vi "Write IFD.vi"(0 "Byte Stream File in":refnum<file>, 1 "Additional Named Tags":cluster{"name":string, "Variant":variant}[](array[cluster]), 2 "Additional Tags":T4(array[cluster]), 3 "byte order (0:big-endian, network order)":T9(ring), 5 "IFD Offset Position":i64 format="%x", 9 "Offset":i64, 11 "error in":errorcluster, 12 "IFD Baseline":T8 {"SampleFormat" items=["UINT"=1, "INT"=2, "FP"=3, "VOID"=4, "COMPLEXINT"=5, "COMPLEXFP"=6]; "NewSubFileType" items=["FILETYPE_REDUCEDIMAGE"=1, "FILETYPE_PAGE"=2, "FILETYPE_MASK"=4]; "Compression" items=["COMPRESSION_NONE"=1, "COMPRESSION_CCITTRLE"=2, "COMPRESSION_CCITTFAX3"=3, "COMPRESSION_CCITTFAX4"=4, "COMPRESSION_LZW"=5, "COMPRESSION_OJPEG"=6, "COMPRESSION_JPEG"=7, "COMPRESSION_NEXT"=32766, "COMPRESSION_CCITTRLEW"=32771, "COMPRESSION_PACKBITS"=32773, "COMPRESSION_THUNDERSCAN"=32809, "COMPRESSION_IT8CTPAD"=32895, "COMPRESSION_IT8LW"=32896, "COMPRESSION_IT8MP"=32897, "COMPRESSION_IT8BL"=32898, "COMPRESSION_PIXARFILM"=32908, "COMPRESSION_PIXARLOG"=32909, "COMPRESSION_DEFLATE"=32946, "COMPRESSION_ADOBE_DEFLATE"=8, "COMPRESSION_DSC"=32947, "COMPRESSION_JBIG"=34661, "COMPRESSION_SGILOG"=34676, "COMPRESSION_SGILOG24"=34677, "COMPRESSION_JP2000"=34712]; "PhotometricInterpretation" items=["PHOTOMETRIC_MINISWHITE"=0, "PHOTOMETRIC_MINISBLACK"=1, "PHOTOMETRIC_RGB"=2, "PHOTOMETRIC_PALETTE"=3, "PHOTOMETRIC_MASK"=4, "PHOTOMETRIC_SEPARATED"=5, "PHOTOMETRIC_YCBCR"=6, "PHOTOMETRIC_CIELAB"=8, "PHOTOMETRIC_ICCLAB"=9, "PHOTOMETRIC_ITULAB"=10, "PHOTOMETRIC_LOGL"=32844, "PHOTOMETRIC_LOGLUV"=32845, "CFA"=32803, "LinearRaw"=34892, "DEPTH"=51177]; "ResolutionUnit" items=["RESUNIT_NONE"=1, "RESUNIT_INCH"=2, "RESUNIT_CENTIMETER"=3]}, 14 "Details":T5={"ImageDescription"="", "XResolution"=0.0, "YResolution"=0.0, "ResolutionUnit"=enum."Inch", "PhotometricInterpretation"=0, "Compression"=enum."None", "PageName"="", "DocumentName"=""} {"PhotometricInterpretation" items=["PHOTOMETRIC_MINISWHITE"=0, "PHOTOMETRIC_MINISBLACK"=1, "PHOTOMETRIC_RGB"=2, "PHOTOMETRIC_PALETTE"=3, "PHOTOMETRIC_MASK"=4, "PHOTOMETRIC_SEPARATED"=5, "PHOTOMETRIC_YCBCR"=6, "PHOTOMETRIC_CIELAB"=8, "PHOTOMETRIC_ICCLAB"=9, "PHOTOMETRIC_ITULAB"=10, "PHOTOMETRIC_LOGL"=32844, "PHOTOMETRIC_LOGLUV"=32845, "CFA"=32803, "LinearRaw"=34892, "DEPTH"=51177]}) -> (4 "refnum out":refnum<file>, 6 "Next IFD Offset Position":i64 format="%x", 10 "Next Offset":i64, 15 "error out":errorcluster)   [LabVIEW 2020, in "LV Tiff.lvlib"]
uses:
  LV Tiff.lvlib
  Baseline Tags 1.ctl
  Tiff Tag.ctl
  Tiff Tags.ctl
  Tiff Data Type.ctl
  Tiff Page Details.ctl
  <vilib>/Utility/Data Type/Type Definitions/Data Type.ctl
  13cce788-e93b-439c-a4f4-f02fbe767664.vi
  de296096-4773-46d0-ada0-82523eb18cea.vi
  <vilib>/Comparison/Less/Less Functor/Less Functor.lvclass
  <vilib>/Utility/Data Type/NI_Data Type.lvlib
panel:
  out "sorted array":T3(array[cluster])
  out "Written Tags":T6[](array[typedef]) {"TagID" items=["NewSubfileType"=254, "ImageWidth"=256, "ImageLength"=257, "BitsPerSample"=258, "Compression"=259, "PhotometricInterpretation"=262, "StripOffsets"=273, "SamplesPerPixel"=277, "RowsPerStrip"=278, "StripByteCounts"=279, "XResolution"=282, "YResolution"=283, "ResolutionUnit"=296, "ColorMap"=320, "PlanarConfiguration"=284, "YCbCrCoefficients"=529, "YCbCrSubSampling"=530, "YCbCrPositioning"=531, "ReferenceBlackWhite"=532, "BadFaxLines"=326, "CleanFaxData"=327, "ConsecutiveBadFaxLines"=328, "SampleFormat"=339]}
  out "This IFD Position":u32
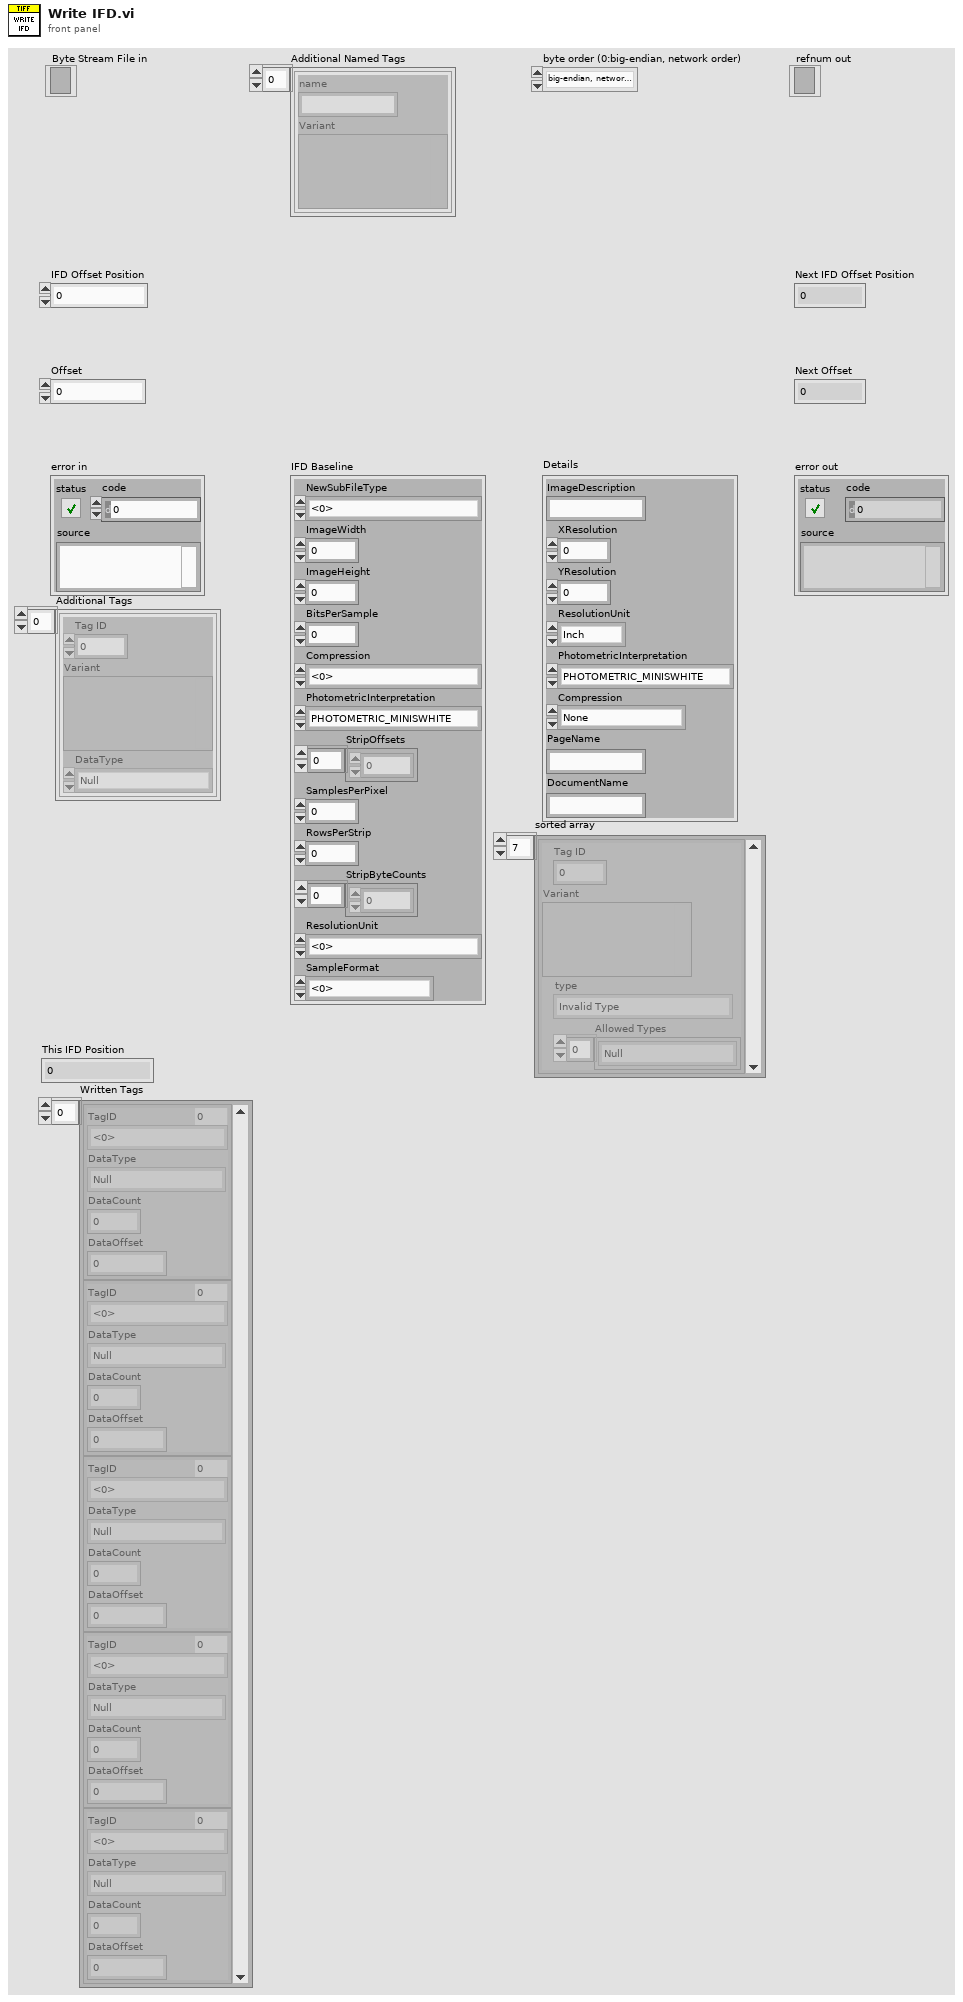
[diagram p1: front panel]
types:
  T1 = typedef "NI_Data Type.lvlib/Data Type.ctl" = enum8{"Invalid Type", "Void", "I8", "I16", "I32", "I64", "U8", "U16", "U32", "U64", "Single Float", "Double Float", "Extended Float", "Single Complex", "Double Complex", "Extended Complex", "Enum U8", "Enum U16", "Enum U32", "Enum U64", "Single Float With Unit", "Double Float With Unit", "Extended Float With Unit", "Single Complex with Unit", "Double Complex with Unit", "Extended Complex with Unit", "Boolean", "String", "Path", "Picture", "Tag", "Array", "Cluster", "Variant", "LV Variant", "Waveform", "Timestamp", "Digital Waveform", "Digital Data", "ExpressData", "Refnum", "External Data", "VI", "Poly VI", "LabVIEW Class Instance", "Fixed Point", "Set Collection", "Map Collection"}
  T2 = typedef "LV Tiff.lvlib/Tiff Data Type.ctl" = enum16{"Null", "BYTE", "ASCII", "SHORT", "LONG", "RATIONAL", "SBYTE", "UNDEFINE", "SSHORT", "SLONG", "SRATIONAL", "FLOAT", "DOUBLE"}
  T3 = cluster{"Tag ID":u32, "Variant":variant, "type":T1, "Allowed Types":T2[]}[]
  T4 = cluster{"Tag ID":u32, "Variant":variant, "DataType":T2}[]
  T5 = typedef "LV Tiff.lvlib/Tiff Page Details.ctl" = cluster{"ImageDescription":string, "XResolution":dbl, "YResolution":dbl, "ResolutionUnit":enum16{"None", "Inch", "Centimeter"}, "PhotometricInterpretation":u16, "Compression":enum16{"None", "Deflate", "JPEG"}, "PageName":string, "DocumentName":string}
  T6 = typedef "LV Tiff.lvlib/Tiff Tag.ctl" = cluster{"TagID":T7, "DataType":T2, "DataCount":u32, "DataOffset":u32}
  T7 = typedef "LV Tiff.lvlib/Tiff Tags.ctl" = u16
  T8 = typedef "LV Tiff.lvlib/Baseline Tags 1.ctl" = cluster{"NewSubFileType":u32, "ImageWidth":u32, "ImageHeight":u32, "BitsPerSample":u16, "Compression":u16, "PhotometricInterpretation":u16, "StripOffsets":u32[], "SamplesPerPixel":u16, "RowsPerStrip":u32, "StripByteCounts":u32[], "ResolutionUnit":u16, "SampleFormat":u16}
  T9 = enum16{"big-endian, network order", "native, host order", "little-endian"}
  T10 = map{string, cluster{"Tag ID":u32, "Allowed Types":T2[]}}
  T11 = cluster{"Tag ID":u32, "Variant":variant, "type":T1, T2[]}
  T12 = cluster{"name":string, "Variant":variant, "type":T1}
  T13 = cluster{"name":string, "Variant":variant, "type":T1}[]
  T14 = cluster{"Tag ID":u32, "Variant":variant, "type":T1, "Allowed Types":T2[]}
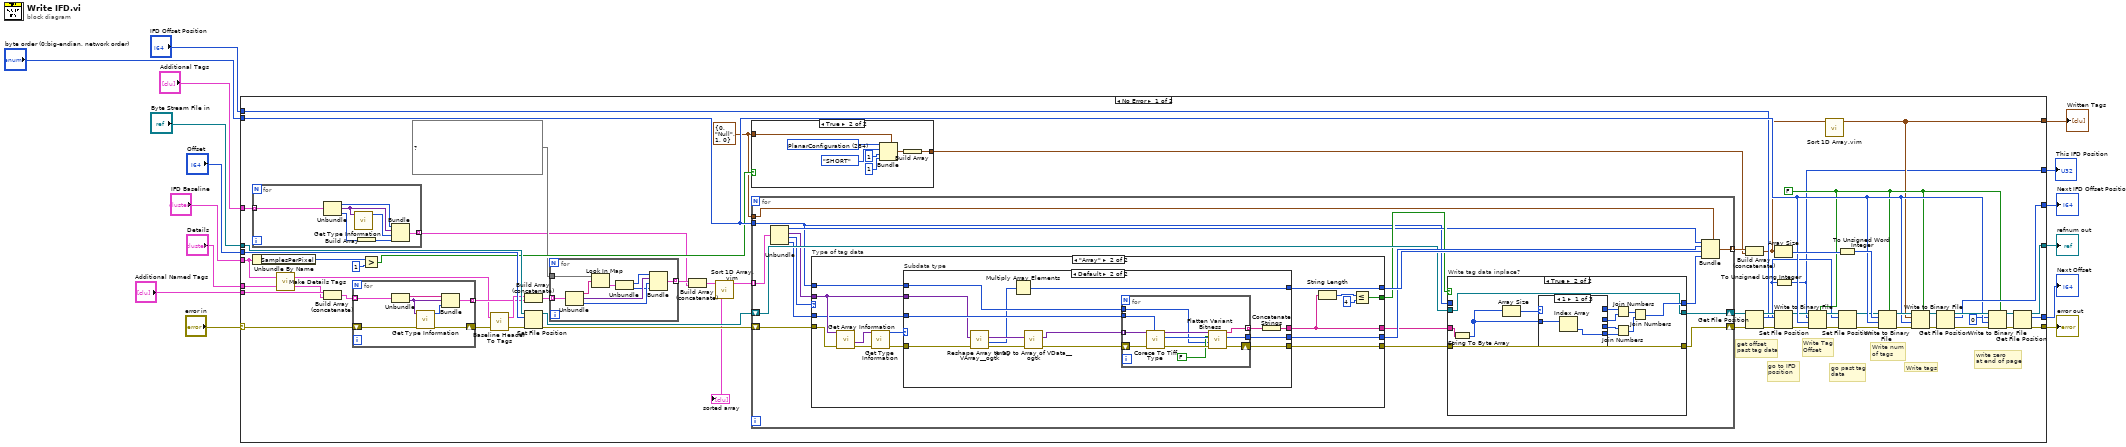
[diagram p0: block diagram]
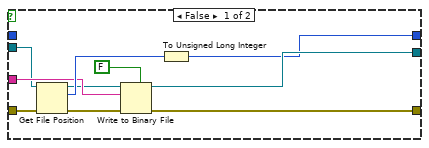
[diagram p3: hidden frame]
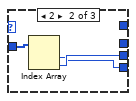
[diagram p4: hidden frame]
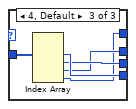
[diagram p5: hidden frame]
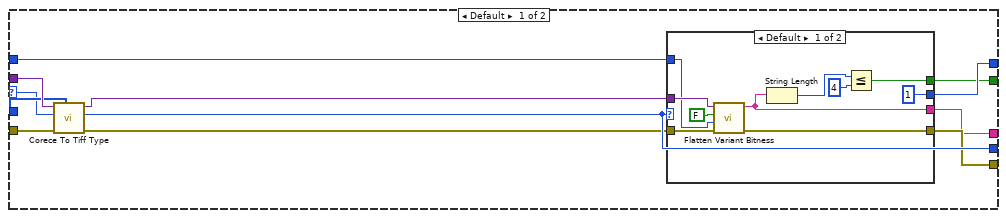
[diagram p6: hidden frame]
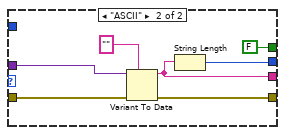
[diagram p7: hidden frame]
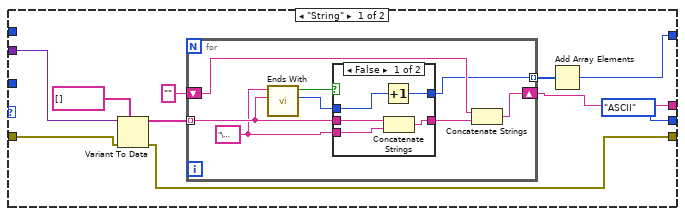
[diagram p8: hidden frame]
diagram:
  n1 = case shown="No Error" "error in" {
    selector: "error in" -> [w38 w250]
    tunnel: "Offset" -> [w75 _]
    tunnel: "Byte Stream File in" -> [w73 w249]
    tunnel: "IFD Baseline" -> [w27 _]
    tunnel: [w63 _] -> w12
    tunnel: [w59 w250] -> w10
    tunnel: [w57 w249] -> w9
    tunnel: [w56 _] -> w8
    tunnel: "byte order (0:big-endian, network order)" -> [w52 _]
    tunnel: "IFD Offset Position" -> [w47 _]
    tunnel: "Additional Named Tags" -> [w40 _]
    tunnel: "Details" -> [w28 _]
    tunnel: "Additional Tags" -> [w22 _]
    tunnel: [w17 _] -> w2
    tunnel: [w16 _] -> w1
    frame No Error {
      w51 = FALSE ("prepend array or string size? (T)")
      w30 = T6 {"TagID"=0, "DataType"=enum."Null", "DataCount"=1, "DataOffset"=0}
      # "write zero\nat end of page"
      # "Write tags"
      # "Write num\nof tags"
      # "go past tag\ndata"
      # "Write Tag\nOffset"
      # "go to IFD position"
      # "get offset\npast tag data"
      n2 = for {
        tunnel: w22 -> [w82] mode=indexing
        tunnel: [w78] -> w21 mode=indexing
        n3 = Unbundle(w82) -> ("Tag ID"=w81:u32, "Variant"=w80:variant, "DataType"=w77:T2)
        n4 = call <vilib>:"Get Type Information.vi"("variant"=w80) -> ("type"=w79:T1)  [unwired: 6 in, 4 out]
        n5 = Build Array(w77) -> (w76:T2[])
        n6 = Bundle("Tag ID"=w81, "Variant"=w80, "type"=w79, w76) -> (w78:T11)  [unwired: 1 in]
      }
      n7 = Unbundle By Name(w27) -> ("SamplesPerPixel"=w33:u16)
      n8 = call "Make Details Tags.vi"("Details"=w28, "IFD Baseline"=w27) -> ("Tags"=w35:cluster{"name":string, "Variant":variant}[], "Modified IFD Baseline"=w26:T8)
      n9 = Build Array (concatenate)(w40, w35) -> (w36:cluster{"name":string, "Variant":variant}[])
      n10 = for {
        tunnel: w36 -> [w105] mode=indexing
        tunnel: [w101] -> w39 mode=indexing
        shift-right: [w99] -> w37
        shift-left: w38 -> [w100]
        n11 = Unbundle(w105) -> ("name"=w104:string, "Variant"=w103:variant)
        n12 = call <vilib>:"Get Type Information.vi"("error in (no error)"=w100, "variant"=w103) -> ("error out"=w99:errorcluster, "type"=w102:T1)  [unwired: 5 in, 3 out]
        n13 = Bundle("name"=w104, "Variant"=w103, "type"=w102) -> (w101:T12)  [unwired: 1 in]
      }
      n14 = Greater?(x=w33, y=u16 1) -> (0:w32:bool)
      n15 = call "Baseline Header To Tags.vi"("error in"=w37, "IFD Baseline"=w26) -> ("error out"=w42:errorcluster, "Tags"=w41:T13)
      n16 = Build Array (concatenate)(w41, w39) -> (w24:T13)
      n17 = Set File Position(offset (in bytes) (0)=w75, refnum=w73, error in=w42) -> (refnum out=w74:refnum<file>, error out=w61:errorcluster)  [unwired: 1 in]
      n18 = for {
        tunnel: T10 {"Artist"={"Tag ID"=315, "Allowed Types"=[enum."ASCII"]}, "BadFaxLines"={"Tag ID"=326, "Allowed Types"=[enum."SHORT", enum."LONG"]}, "BitsPerSample"={"Tag ID"=258, "Allowed Types"=[enum."SHORT"]}, "BlackIsZero"={"Tag ID"=1, "Allowed Types"=[]}, "CCITT 1D"={"Tag ID"=2, "Allowed Types"=[]}, "CCITT Group 3"={"Tag ID"=3, "Allowed Types"=[]}, "CCITT Group 4"={"Tag ID"=4, "Allowed Types"=[]}, "CIELab"={"Tag ID"=8, "Allowed Types"=[]}, "CMYK"={"Tag ID"=5, "Allowed Types"=[]}, "CellLength"={"Tag ID"=265, "Allowed Types"=[enum."SHORT"]}, "CellWidth"={"Tag ID"=264, "Allowed Types"=[enum."SHORT"]}, "CleanFaxData"={"Tag ID"=327, "Allowed Types"=[enum."SHORT"]}, "ColorMap"={"Tag ID"=320, "Allowed Types"=[enum."SHORT"]}, "ColorResponseCurve"={"Tag ID"=301, "Allowed Types"=[enum."SHORT"]}, "ColorResponseUnit"={"Tag ID"=300, "Allowed Types"=[enum."SHORT"]}, "Compression"={"Tag ID"=259, "Allowed Types"=[enum."SHORT"]}, "ConsecutiveBadFaxLines"={"Tag ID"=328, "Allowed Types"=[enum."LONG", enum."SHORT"]}, "Copyright"={"Tag ID"=33432, "Allowed Types"=[enum."ASCII"]}, "DateTime"={"Tag ID"=306, "Allowed Types"=[enum."ASCII"]}, "DocumentName"={"Tag ID"=269, "Allowed Types"=[enum."ASCII"]}, "DotRange"={"Tag ID"=336, "Allowed Types"=[enum."BYTE", enum."SHORT"]}, "ExtraSamples"={"Tag ID"=338, "Allowed Types"=[enum."BYTE"]}, "FillOrder"={"Tag ID"=266, "Allowed Types"=[enum."SHORT"]}, "FreeByteCounts"={"Tag ID"=289, "Allowed Types"=[enum."LONG"]}, "FreeOffsets"={"Tag ID"=288, "Allowed Types"=[enum."LONG"]}, "GrayResponseCurve"={"Tag ID"=291, "Allowed Types"=[enum."SHORT"]}, "GrayResponseUnit"={"Tag ID"=290, "Allowed Types"=[enum."SHORT"]}, "HalftoneHints"={"Tag ID"=321, "Allowed Types"=[enum."SHORT"]}, "HostComputer"={"Tag ID"=316, "Allowed Types"=[enum."ASCII"]}, "ImageDescription"={"Tag ID"=270, "Allowed Types"=[enum."ASCII"]}, "ImageHeight"={"Tag ID"=257, "Allowed Types"=[enum."SHORT", enum."LONG"]}, "ImageWidth"={"Tag ID"=256, "Allowed Types"=[enum."SHORT", enum."LONG"]}, "InkNames"={"Tag ID"=333, "Allowed Types"=[enum."ASCII"]}, "InkSet"={"Tag ID"=332, "Allowed Types"=[enum."SHORT"]}, "JPEG"={"Tag ID"=6, "Allowed Types"=[]}, "JPEGACTTables"={"Tag ID"=521, "Allowed Types"=[enum."LONG"]}, "JPEGDCTTables"={"Tag ID"=520, "Allowed Types"=[enum."LONG"]}, "JPEGInterchangeFormat"={"Tag ID"=513, "Allowed Types"=[enum."LONG"]}, "JPEGInterchangeFormatLength"={"Tag ID"=514, "Allowed Types"=[enum."LONG"]}, "JPEGLosslessPredictors"={"Tag ID"=517, "Allowed Types"=[enum."SHORT"]}, "JPEGPointTransforms"={"Tag ID"=518, "Allowed Types"=[enum."SHORT"]}, "JPEGProc"={"Tag ID"=512, "Allowed Types"=[enum."SHORT"]}, "JPEGQTables"={"Tag ID"=519, "Allowed Types"=[enum."LONG"]}, "JPEGRestartInterval"={"Tag ID"=515, "Allowed Types"=[enum."SHORT"]}, "LZW"={"Tag ID"=5, "Allowed Types"=[]}, "Make"={"Tag ID"=271, "Allowed Types"=[enum."ASCII"]}, "MaxSampleValue"={"Tag ID"=281, "Allowed Types"=[enum."SHORT"]}, "MinSampleValue"={"Tag ID"=280, "Allowed Types"=[enum."SHORT"]}, "Model"={"Tag ID"=272, "Allowed Types"=[enum."ASCII"]}, "NewSubFileType"={"Tag ID"=254, "Allowed Types"=[enum."LONG"]}, "NumberOfInks"={"Tag ID"=334, "Allowed Types"=[enum."SHORT"]}, "Orientation"={"Tag ID"=274, "Allowed Types"=[enum."SHORT"]}, "Packbits"={"Tag ID"=32773, "Allowed Types"=[]}, "PageName"={"Tag ID"=285, "Allowed Types"=[enum."ASCII"]}, "PageNumber"={"Tag ID"=297, "Allowed Types"=[enum."SHORT"]}, "PhotometricInterpretation"={"Tag ID"=262, "Allowed Types"=[enum."SHORT"]}, "PlanarConfiguration"={"Tag ID"=284, "Allowed Types"=[enum."SHORT"]}, "Predictor"={"Tag ID"=317, "Allowed Types"=[enum."SHORT"]}, "PrimaryChromaticities"={"Tag ID"=319, "Allowed Types"=[enum."RATIONAL"]}, "RGB"={"Tag ID"=2, "Allowed Types"=[]}, "RGB Palette"={"Tag ID"=3, "Allowed Types"=[]}, "ReferenceBlackWhite"={"Tag ID"=532, "Allowed Types"=[enum."LONG"]}, "ResolutionUnit"={"Tag ID"=296, "Allowed Types"=[enum."SHORT"]}, "RowsPerStrip"={"Tag ID"=278, "Allowed Types"=[enum."SHORT", enum."LONG"]}, "SMaxSampleValue"={"Tag ID"=341, "Allowed Types"=[enum."Null"]}, "SMinSampleValue"={"Tag ID"=340, "Allowed Types"=[enum."Null"]}, "SampleFormat"={"Tag ID"=339, "Allowed Types"=[enum."SHORT"]}, "SamplesPerPixel"={"Tag ID"=277, "Allowed Types"=[enum."SHORT"]}, "Software"={"Tag ID"=305, "Allowed Types"=[enum."ASCII"]}, "StripByteCounts"={"Tag ID"=279, "Allowed Types"=[enum."LONG", enum."SHORT"]}, "StripOffsets"={"Tag ID"=273, "Allowed Types"=[enum."SHORT", enum."LONG"]}, "SubFileType"={"Tag ID"=255, "Allowed Types"=[enum."SHORT"]}, "T4Options[2]"={"Tag ID"=292, "Allowed Types"=[enum."LONG"]}, "T6Options[3]"={"Tag ID"=293, "Allowed Types"=[enum."LONG"]}, "TargetPrinter"={"Tag ID"=337, "Allowed Types"=[enum."ASCII"]}, "Thresholding"={"Tag ID"=263, "Allowed Types"=[enum."SHORT"]}, "TileByteCounts"={"Tag ID"=325, "Allowed Types"=[enum."SHORT", enum."LONG"]}, "TileLength"={"Tag ID"=323, "Allowed Types"=[enum."SHORT", enum."LONG"]}, "TileOffsets"={"Tag ID"=324, "Allowed Types"=[enum."LONG"]}, "TileWidth"={"Tag ID"=322, "Allowed Types"=[enum."SHORT", enum."LONG"]}, "Tranparency Mask"={"Tag ID"=4, "Allowed Types"=[]}, "TransferFunction[4]"={"Tag ID"=301, "Allowed Types"=[enum."SHORT"]}, "TransferRange"={"Tag ID"=342, "Allowed Types"=[enum."SHORT"]}, "Uncompressed"={"Tag ID"=32771, "Allowed Types"=[]}, "WhiteIsZero"={"Tag ID"=0, "Allowed Types"=[]}, "WhitePoint"={"Tag ID"=318, "Allowed Types"=[enum."RATIONAL"]}, "XPosition"={"Tag ID"=286, "Allowed Types"=[enum."RATIONAL"]}, "XResolution"={"Tag ID"=282, "Allowed Types"=[enum."RATIONAL"]}, "YCbCr"={"Tag ID"=6, "Allowed Types"=[]}, "YCbCrCoefficients"={"Tag ID"=529, "Allowed Types"=[enum."RATIONAL"]}, "YCbCrPositioning"={"Tag ID"=531, "Allowed Types"=[enum."SHORT"]}, "YCbCrSubSampling"={"Tag ID"=530, "Allowed Types"=[enum."SHORT"]}, "YPosition"={"Tag ID"=287, "Allowed Types"=[enum."RATIONAL"]}, "YResolution"={"Tag ID"=283, "Allowed Types"=[enum."RATIONAL"]}} ("Map") -> [w91]
        tunnel: w24 -> [w90] mode=indexing
        tunnel: [w83] -> w23 mode=indexing
        n19 = Unbundle(w90) -> ("name"=w87:string, "Variant"=w86:variant, "type"=w85:T1)
        n20 = Look In Map(map=w91, key=w87) -> (value=w89:cluster{"Tag ID":u32, "Allowed Types":T2[]})  [unwired: 1 in, 1 out]
        n21 = Unbundle(w89) -> ("Tag ID"=w88:u32, "Allowed Types"=w84:T2[])
        n22 = Bundle("Tag ID"=w88, "Variant"=w86, "type"=w85, "Allowed Types"=w84) -> (w83:T14)  [unwired: 1 in]
      }
      n23 = Build Array (concatenate)(w23, w21) -> (w19:T3)
      n24 = call "Sort 1D Array.vim"("unsorted array"=w19) -> ("sorted array"=w18:T3)  [unwired: 10 in]
      "sorted array" <- w18
      n25 = case shown="True" w32 {
        tunnel: w30 -> [_ w98]
        tunnel: [_ w92] -> w29
        frame False {
        }
        frame True {
          w97 = T7 284 items=["NewSubfileType"=254, "ImageWidth"=256, "ImageLength"=257, "BitsPerSample"=258, "Compression"=259, "PhotometricInterpretation"=262, "StripOffsets"=273, "SamplesPerPixel"=277, "RowsPerStrip"=278, "StripByteCounts"=279, "XResolution"=282, "YResolution"=283, "ResolutionUnit"=296, "ColorMap"=320, "PlanarConfiguration"=284, "YCbCrCoefficients"=529, "YCbCrSubSampling"=530, "YCbCrPositioning"=531, "ReferenceBlackWhite"=532, "BadFaxLines"=326, "CleanFaxData"=327, "ConsecutiveBadFaxLines"=328, "SampleFormat"=339] ("Ring")
          n26 = Bundle(cluster=w98, "TagID"=w97, "DataType"=Tiff_Data_Type."SHORT", "DataCount"=u32 1, "DataOffset"=u32 1) -> (w93:T6)
          n27 = Build Array(w93) -> (w92:T6[])
        }
      }
      n28 = for {
        tunnel: w30 -> [w123]
        shift-right: [w120] -> w54
        shift-left: w74 -> [w119]
        tunnel: w52 -> [w106]
        tunnel: [w107] -> w72 mode=indexing
        shift-right: [w115] -> w62
        shift-left: w61 -> [w113]
        tunnel: w18 -> [w112] mode=indexing
        n29 = Unbundle(w112) -> ("Tag ID"=w109:u32, "Variant"=w110:variant, "type"=w111:T1, "Allowed Types"=w108:T2[])
        n30 = case "Type of tag data" shown="\"Array\"" w111 {
          selector: w111 -> [w157 _]
          tunnel: w110 -> [w167 w195]
          tunnel: [w163 w199] -> w122
          tunnel: [w164 w196] -> w121
          tunnel: [w158 w189] -> w116
          tunnel: [w160 w186] -> w117
          tunnel: w113 -> [w166 w194]
          tunnel: [w161 w191] -> w114
          tunnel: w108 -> [w165 w190]
          tunnel: w106 -> [w156 w185]
          frame Default {
            n31 = call "Corece To Tiff Type.vi"("Allowed Types"=w165, "error in (no error)"=w166, "Variant Data type (optional)"=w157, "Variant"=w167) -> ("error out"=w162:errorcluster, "Actual Type"=w164:T2, "Coerced Variant"=w159:variant)  [unwired: 5 in]
            n32 = case shown="Default" w164 {
              tunnel: [u32 1 ("Size") w179] -> w163
              tunnel: w162 -> [w171 w184]
              tunnel: [w170 w183] -> w161
              tunnel: [w175 FALSE] -> w160
              tunnel: w159 -> [w173 w182]
              tunnel: [w172 w180] -> w158
              tunnel: w156 -> [w168 _]
              frame Default {
                n33 = call "Flatten Variant Bitness.vi"("error in (no error)"=w171, "byte order (0:big-endian, network order)"=w168, "Prepend Array or String size (T)"=FALSE, "Variant"=w173) -> ("error out"=w170:errorcluster, "data string"=w172:string)  [unwired: 6 in]
                n34 = String Length(string=w172) -> (length=w174:i32)
                n35 = Less Or Equal?(x=w174, y=4) -> (x <= y?=w175:bool)
              }
              frame "ASCII" {
                n36 = Variant To Data(error in=w184, type="", Variant=w182) -> (data=w180:string, error out=w183:errorcluster)
                n37 = String Length(string=w180) -> (length=w179:i32)
              }
            }
          }
          frame "Array" {
            n38 = call <vilib>:"Get Array Information.vi"("error in (no error)"=w194, "variant"=w195) -> ("error out"=w193:errorcluster, "array element data type"=w198:variant)  [unwired: 6 in, 2 out]
            n39 = call <vilib>:"Get Type Information.vi"("error in (no error)"=w193, "variant"=w198) -> ("error out"=w192:errorcluster, "type"=w197:T1)  [unwired: 5 in, 3 out]
            n40 = case "Subdata type" shown="Default" w197 {
              tunnel: [w204 w226] -> w199
              tunnel: [w202 w235] -> w189
              tunnel: [Tiff_Data_Type."ASCII" ("DataType") w236] -> w196
              tunnel: w195 -> [w209 w231]
              tunnel: w192 -> [w201 w232]
              tunnel: [w200 w238] -> w191
              tunnel: w190 -> [_ w237]
              tunnel: w185 -> [_ w233]
              frame "String" {
                n41 = Variant To Data(error in=w201, type=string[] [], Variant=w209) -> (data=w207:string[], error out=w200:errorcluster)
                n42 = for {
                  tunnel: w207 -> [w216] mode=indexing
                  shift-right: [w213] -> w202
                  shift-left: "" -> [w214]
                  tunnel: [w211] -> w205 mode=indexing
                  w215 = "\u0000" ("Suffix")
                  n43 = call "Ends With.vi"("String"=w216, "Suffix"=w215) -> ("String length"=w210:i32, "Ended with"=w217:bool)  [unwired: 8 in]
                  n44 = case shown="False" w217 {
                    tunnel: [w221 w224] -> w212
                    tunnel: w216 -> [w222 w224]
                    tunnel: w215 -> [w220 _]
                    tunnel: [w218 w223] -> w211
                    tunnel: w210 -> [w219 w223]
                    frame False {
                      n45 = Increment(x=w219) -> (x+1=w218:i32)
                      n46 = Concatenate Strings(w222, w220) -> (w221:string)
                    }
                    frame True {
                    }
                  }
                  n47 = Concatenate Strings(w214, w212) -> (w213:string)
                }
                n48 = Add Array Elements(numeric array=w205) -> (sum=w204:i32)
              }
              frame Default {
                n49 = call <userlib>:"Reshape Array to 1D VArray__ogtk.vi"("error in (no error)"=w232, "MultiD Array"=w231) -> ("error out"=w230:errorcluster, "Size(s)"=w227:u32[], "1D VArray"=w229:variant)  [unwired: 7 in]
                n50 = Multiply Array Elements(1:w227) -> (0:w226:u32)
                n51 = call <userlib>:"Array to Array of VData__ogtk.vi"("error in (no error)"=w230, "MultiD Array"=w229) -> ("error out"=w228:errorcluster, "1D Array of Variants"=w225:variant[])  [unwired: 8 in]
                n52 = for {
                  tunnel: w225 -> [w247] mode=indexing
                  shift-right: [w242] -> w238
                  shift-left: w228 -> [w248]
                  tunnel: w237 -> [w246]
                  tunnel: [w245] -> w236
                  tunnel: [w241] -> w234 mode=indexing
                  tunnel: w233 -> [w239]
                  n53 = call "Corece To Tiff Type.vi"("Allowed Types"=w246, "error in (no error)"=w248, "Variant"=w247) -> ("error out"=w243:errorcluster, "Actual Type"=w245:T2, "Coerced Variant"=w244:variant)  [unwired: 6 in]
                  n54 = call "Flatten Variant Bitness.vi"("error in (no error)"=w243, "byte order (0:big-endian, network order)"=w239, "Prepend Array or String size (T)"=FALSE, "Variant"=w244) -> ("error out"=w242:errorcluster, "data string"=w241:string)  [unwired: 6 in]
                }
                n55 = Concatenate Strings(w234) -> (w235:string)
              }
            }
            n56 = String Length(string=w189) -> (length=w188:i32)
            n57 = Less Or Equal?(x=w188, y=4) -> (x <= y?=w186:bool)
          }
        }
        n58 = case "Write tag data inplace?" shown="True" w117 {
          tunnel: [w125 w134] -> w120
          tunnel: w119 -> [w130 w134]
          tunnel: w116 -> [w131 w145]
          tunnel: [w124 w137] -> w118
          tunnel: w106 -> [_ _]
          tunnel: [w126 w138] -> w115
          tunnel: w114 -> [w128 w138]
          frame False {
            n59 = Get File Position(4:w128, 7:w130) -> (0:w127:errorcluster, 2:w132:i64, 3:w129:refnum<file>)
            n60 = Write to Binary File(file (use dialog)=w129, data=w131, error in=w127, 5:FALSE ("prepend array or string size? (T)")) -> (refnum out=w125:refnum<file>, error out=w126:errorcluster)  [unwired: 2 in, 1 out]
            n61 = To Unsigned Long Integer(number=w132) -> (unsigned 32bit integer=w124:u32)
          }
          frame True {
            n62 = String To Byte Array(string=w145) -> (unsigned byte array=w136:u8[])
            n63 = Array Size(array=w136) -> (size(s)=w135:i32)
            n64 = case shown="1" w135 {
              tunnel: [_ _ w151] -> w144
              tunnel: [_ _ w152] -> w143
              tunnel: [_ w149 w153] -> w142
              tunnel: [w146 w148 w154] -> w141
              tunnel: w136 -> [w147 w150 w155]
              frame 1 {
                n65 = Index Array(array=w147) -> (element=w146:u8)  [unwired: 1 in]
              }
              frame 2 {
                n66 = Index Array(array=w150) -> (element #1=w148:u8, element #2=w149:u8)  [unwired: 2 in]
              }
              frame 4, Default {
                n67 = Index Array(array=w155) -> (element #1=w154:u8, element #2=w153:u8, element #3=w152:u8, element #4=w151:u8)  [unwired: 4 in]
              }
            }
            n68 = Join Numbers(hi=w144, lo=w143) -> ((hi.lo)=w140:u16)
            n69 = Join Numbers(hi=w142, lo=w141) -> ((hi.lo)=w139:u16)
            n70 = Join Numbers(hi=w140, lo=w139) -> ((hi.lo)=w137:u32)
          }
        }
        n71 = Bundle(cluster=w123, "TagID"=w109, "DataType"=w121, "DataCount"=w122, "DataOffset"=w118) -> (w107:T6)
      }
      n72 = Build Array (concatenate)(w72, w29) -> (w34:T6[])
      n73 = Get File Position(4:w62, 7:w54) -> (0:w55:errorcluster, 2:w43:i64, 3:w49:refnum<file>)
      n74 = Array Size(array=w34) -> (size(s)=w71:i32)
      n75 = To Unsigned Long Integer(number=w43) -> (unsigned 32bit integer=w16:u32)
      n76 = Set File Position(offset (in bytes) (0)=w47, refnum=w49, error in=w55) -> (refnum out=w48:refnum<file>, error out=w50:errorcluster)  [unwired: 1 in]
      n77 = Write to Binary File(file (use dialog)=w48, data=w16, error in=w50, 5:w51, 9:w52) -> (refnum out=w45:refnum<file>, error out=w53:errorcluster)  [unwired: 1 in, 1 out]
      n78 = call "Sort 1D Array.vim"("unsorted array"=w34) -> ("sorted array"=w17:T6[])  [unwired: 10 in]
      n79 = To Unsigned Word Integer(number=w71) -> (unsigned 16bit integer=w70:u16)
      n80 = Set File Position(offset (in bytes) (0)=w43, refnum=w45, error in=w53) -> (refnum out=w44:refnum<file>, error out=w46:errorcluster)  [unwired: 1 in]
      n81 = Write to Binary File(file (use dialog)=w44, data=w70, error in=w46, 5:w51, 9:w52) -> (refnum out=w68:refnum<file>, error out=w69:errorcluster)  [unwired: 1 in, 1 out]
      n82 = Write to Binary File(file (use dialog)=w68, data=w17, error in=w69, 5:w51, 9:w52) -> (refnum out=w65:refnum<file>, error out=w67:errorcluster)  [unwired: 1 in, 1 out]
      n83 = Get File Position(4:w67, 7:w65) -> (0:w66:errorcluster, 2:w63:i64, 3:w64:refnum<file>)
      n84 = Write to Binary File(file (use dialog)=w64, data=u32 0, error in=w66, 5:w51, 9:w52) -> (refnum out=w58:refnum<file>, error out=w60:errorcluster)  [unwired: 1 in, 1 out]
      n85 = Get File Position(4:w60, 7:w58) -> (0:w59:errorcluster, 2:w56:i64, 3:w57:refnum<file>)
    }
    frame Error {
    }
  }
  "Next IFD Offset Position" <- w12
  "refnum out" <- w9
  "error out" <- w10
  "Next Offset" <- w8
  "Written Tags" <- w2
  "This IFD Position" <- w1
